vi "PropertyMerge.vi"   [LabVIEW 2023, in "REVLibDriver.lvlib"]
uses:
  <vilib>/REVLibDriver/REVLibDriver.lvlib
  <resource>/objmgr/REVSpark.rc
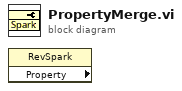
[diagram p0: block diagram]
diagram:
  n1 = property class="RevSpark" props=[]() -> ()  [unwired: 2 in, 3 out]
